vi "Main.vi"() -> ()   [LabVIEW 2026]
doc: "This Continuous Measurement sample project is based on the Queued Message Handler template.\n\nThe Event Handling Loop generates messages based on user interface actions.\n\nThe Message Handling Loop processes messages generated by the Event Handling Loop, or by other messages. There are also Acquisition and Logging message handling loop subVIs, and a chart updating loop."
uses:
  Settings/Settings.ctl
  Acquisition/Hardware Configuration.ctl
  Acquisition/Signal Type.ctl
  Logging/Logging Configuration.ctl
  controls/UI Data.ctl
  controls/UI State.ctl
  support/Message Queue/Enqueue Message (Single).vi
  support/Message Queue/Enqueue Message (Array).vi
  <vilib>/Utility/error.llb/Error Cluster From Error Code.vi
  <vilib>/ErrorRing/Error Ring.xnode
  Acquisition/Acquisition.lvlib
  Logging/Logging.lvlib
  Settings/Settings.lvlib
  support/User Event - Stop/User Event - Stop.lvlib
  support/Message Queue/Message Queue.lvlib
  Settings/Settings Dialog.vi
panel:
  out "Data":waveform(dbl)[](graph)
  in  "Settings":bool
  in  "Start":bool
  in  "Stop":bool
  out "Status":string
  in  "Exit":bool
  # "Continuous Measurement Data Logger"
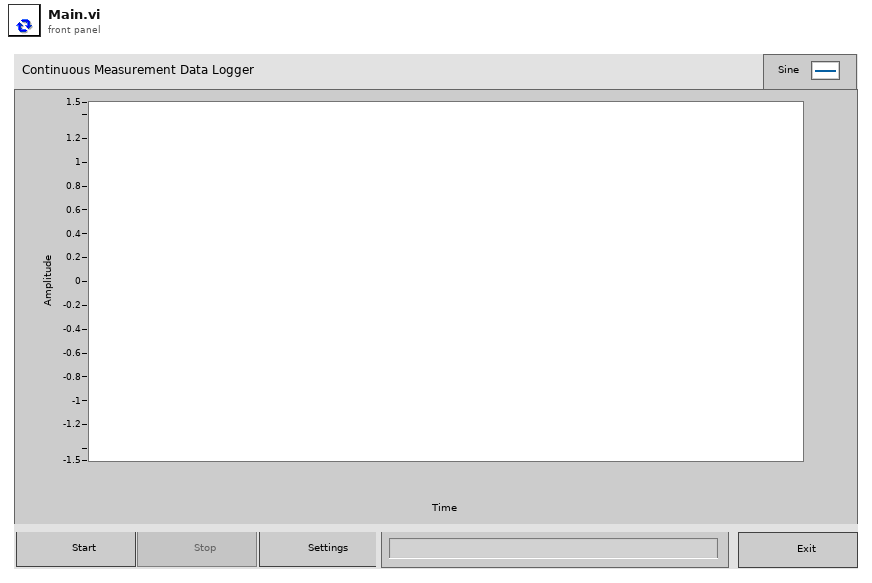
[diagram p1: front panel]
types:
  T1 = typedef "UI State.ctl" = enum16{"Idle", "Acquiring and Logging", "Waiting for Exit", "Waiting for Exit (Acq Stopped)", "Waiting for Exit (Log Stopped)", "Waiting for Stop", "Waiting for Stop (Acq Stopped)", "Waiting for Stop (Log Stopped)"}
  T2 = typedef "UI Data.ctl" = cluster{"Start Ref":refnum<vi>, "Stop Ref":refnum<vi>, "Settings Ref":refnum<vi>, "Exit Ref":refnum<vi>, "Status Ref":refnum<vi>, "Data Ref":refnum<vi>}
  T3 = typedef "Settings.lvlib/Settings.ctl" = cluster{"Hardware Configuration":T4, "Logging Configuration":T6}
  T4 = typedef "Acquisition.lvlib/Hardware Configuration.ctl" = cluster{"HW Refnum <Replace Me>":string, "Signal Type <Replace Me>":T5}
  T5 = typedef "Acquisition.lvlib/Signal Type.ctl" = enum16{"Sine Wave", "Square with Noise"}
  T6 = typedef "Logging.lvlib/Logging Configuration.ctl" = cluster{"Log File Base Path":path, "TDMS File Reference":refnum<k34>}
  T7 = typedef "Message Queue.lvlib/All Message Queues.ctl" = cluster{"UI":refnum<queue>, "Acquisition":refnum<queue>, "Logging":refnum<queue>}
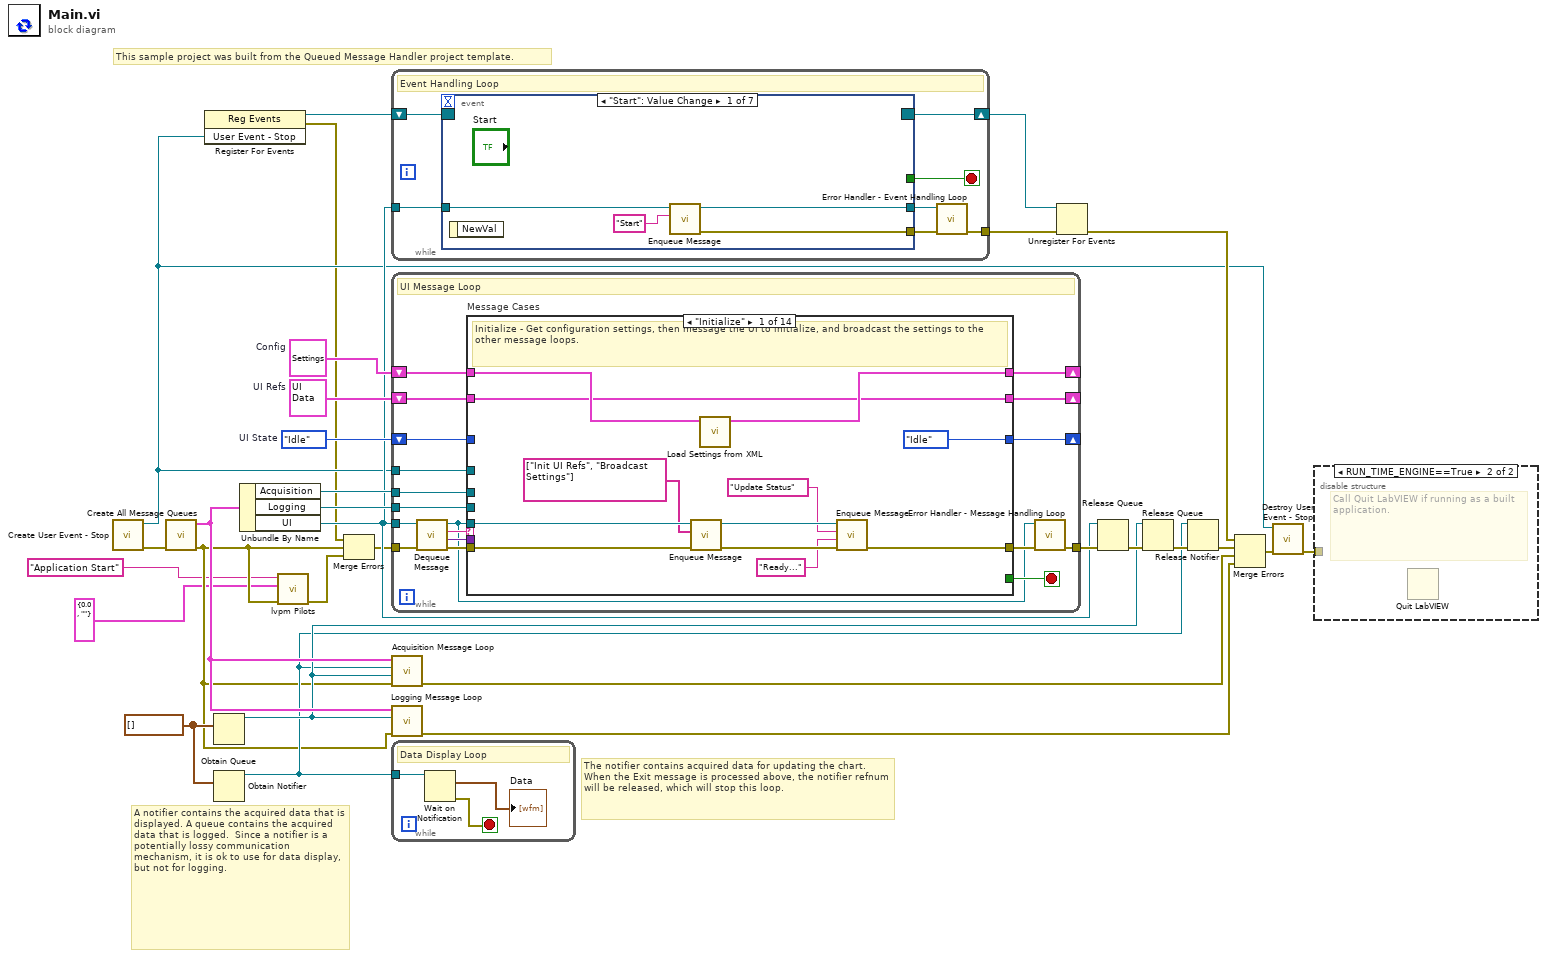
[diagram p0: block diagram]
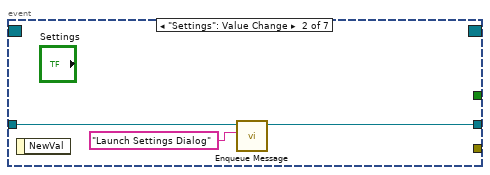
[diagram p3: hidden frame]
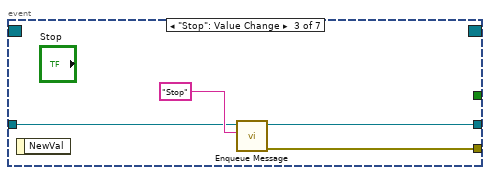
[diagram p4: hidden frame]
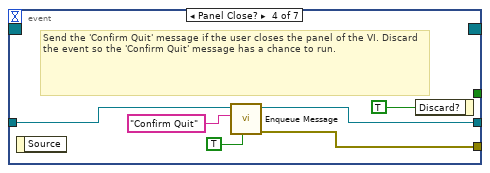
[diagram p5: hidden frame]
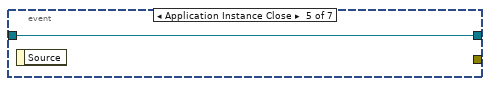
[diagram p6: hidden frame]
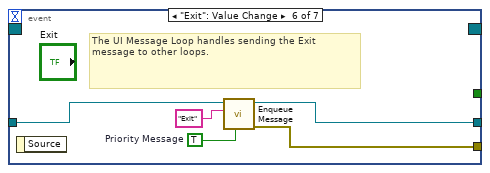
[diagram p7: hidden frame]
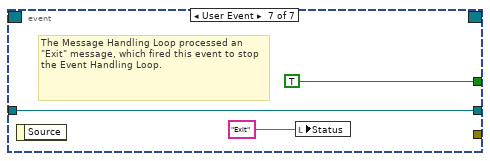
[diagram p8: hidden frame]
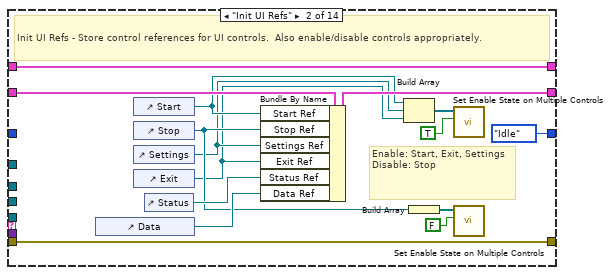
[diagram p9: hidden frame]
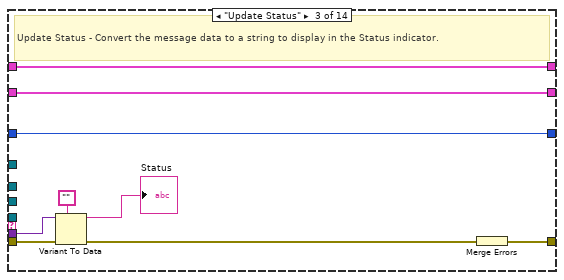
[diagram p10: hidden frame]
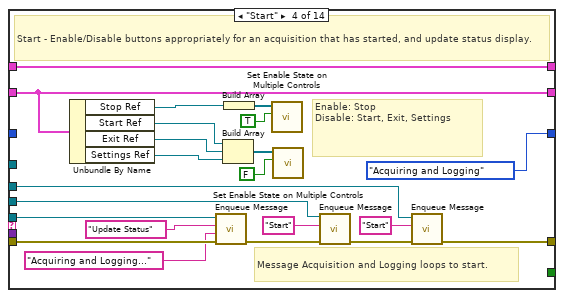
[diagram p11: hidden frame]
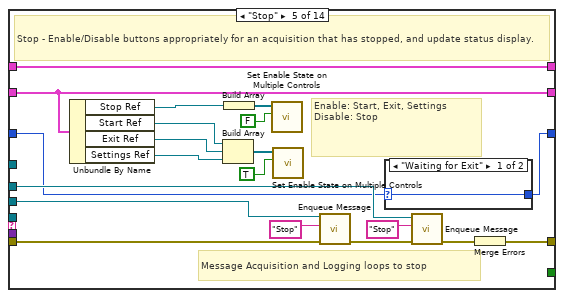
[diagram p12: hidden frame]
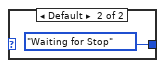
[diagram p13: hidden frame]
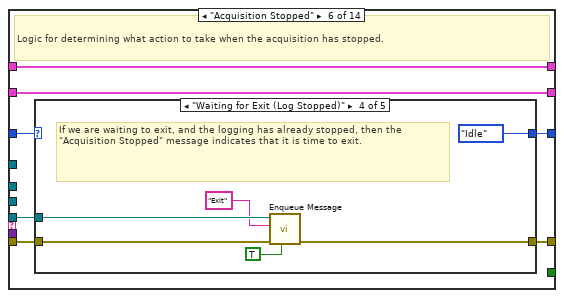
[diagram p14: hidden frame]
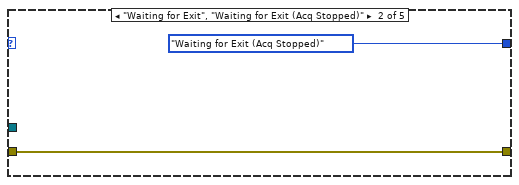
[diagram p16: hidden frame]
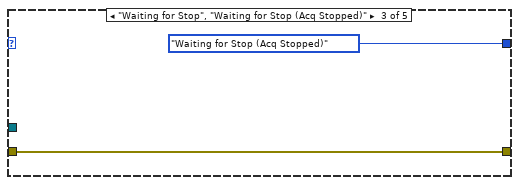
[diagram p17: hidden frame]
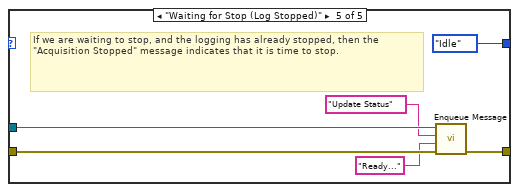
[diagram p18: hidden frame]
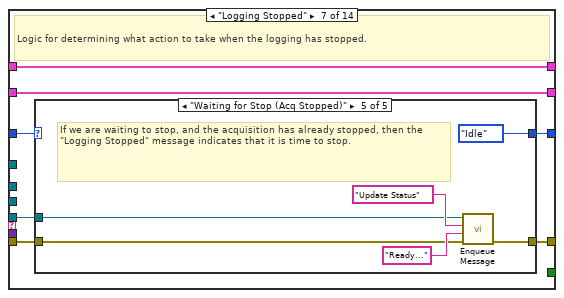
[diagram p19: hidden frame]
diagram:
  w18 = UI_State."Idle"  # UI State
  w9 = waveform(dbl)[] []
  w21 = T2 {"Start Ref"=refnum, "Stop Ref"=refnum, "Settings Ref"=refnum, "Exit Ref"=refnum, "Status Ref"=refnum, "Data Ref"=refnum}  # UI Refs
  w24 = T3 {"Hardware Configuration"={"HW Refnum <Replace Me>"="", "Signal Type <Replace Me>"=enum."Sine Wave"}, "Logging Configuration"={"Log File Base Path"=path "", "TDMS File Reference"=refnum}}  # Config
  # "This sample project was built from the Queued Message Handler project template."
  # "A notifier contains the acquired data that is displayed. A queue contains the acquired data that is logged.  Since a notifier is a potentially lossy communication mechanism, it is ok to use for data display, but not for logging."
  # "The notifier contains acquired data for updating the chart. When the Exit message is processed above, the notifier refnum will be released, which will stop this loop."
  n1 = call "Create User Event - Stop.vi"() -> ("error out"=w27:errorcluster, "User Event - Stop"=w7:refnum<user-event>)  [unwired: 10 in]
  n2 = call "Create All Message Queues.vi"("error in (no error)"=w27) -> ("error out"=w4:errorcluster, "Message Queues out"=w26:T7)  [unwired: 9 in]
  n3 = register-events(w7) -> (reference out=w8:refnum<event-registration>, error out=w5:errorcluster)  [unwired: 2 in]
  n4 = Obtain Queue(element data type=w9) -> (queue out=w11:refnum<queue>)  [unwired: 4 in, 2 out]
  n5 = Obtain Notifier(notification data type=w9) -> (notifier out=w10:refnum<notifier>)  [unwired: 3 in, 2 out]
  n6 = Unbundle By Name(w26) -> ("Acquisition"=w20:refnum<queue>, "Logging"=w19:refnum<queue>, "UI"=w16:refnum<queue>)
  n7 = call "lvpm Pilots.vi"("error in"=w4, "settings"=cluster{"rate (Hz)":dbl, "channel":string} {"rate (Hz)"=0.0, "channel"=""}, "message"="Application Start") -> ("error out"=w1:errorcluster)  [unwired: 7 in, 1 out]
  n8 = Merge Errors(w5, w4, w1) -> (w6:errorcluster)
  n9 = while {
    tunnel: w16 -> [w36]
    tunnel: [w33] -> w29
    shift-right: [w35] -> w22
    shift-left: w8 -> [w37]
    stop <- w34 stop-if-true
    # "Event Handling Loop"
    n10 = event shown="[0] \"Start\": Value Change" {
      selector: w37 -> [_ _ _ _ _ _ _]
      dyn-events: [_ _ _ _ _ _ _] -> w35
      timeout: _ -> [_ _ _ _ _ _ _]
      tunnel: [_ _ _ _ _ _ TRUE ("Discard?")] -> w34
      tunnel: w36 -> [w41 w43 w47 w52 w55 w57 w61]
      tunnel: [w39 _ w46 w50 _ w60 _] -> w32
      tunnel: [w38 w42 w45 w51 w55 w56 w61] -> w31
      event "Start": Value Change {
        n11 = event-data() -> ()  [unwired: 1 in, 1 out]
        n12 = call-poly "Enqueue Message.vi"("Message"="Start", "Message Queue"=w41) -> ("error out"=w39:errorcluster, "dup Message Queue"=w38:refnum<queue>)  [unwired: 8 in]
      }
      event "Settings": Value Change {
        n13 = event-data() -> ()  [unwired: 1 in, 1 out]
        n14 = call-poly "Enqueue Message.vi"("Message"="Launch Settings Dialog", "Message Queue"=w43) -> ("dup Message Queue"=w42:refnum<queue>)  [unwired: 8 in, 1 out]
      }
      event "Stop": Value Change {
        n15 = event-data() -> ()  [unwired: 1 in, 1 out]
        n16 = call-poly "Enqueue Message.vi"("Message"="Stop", "Message Queue"=w47) -> ("error out"=w46:errorcluster, "dup Message Queue"=w45:refnum<queue>)  [unwired: 8 in]
      }
      event Panel Close? {
        # "Send the 'Confirm Quit' message if the user closes the panel of the VI. Discard the event so the 'Confirm Quit' message has a chance to run."
        n17 = event-data() -> ()  [unwired: 1 in, 1 out]
        n18 = call-poly "Enqueue Message.vi"("Priority Message? (F)"=TRUE, "Message"="Confirm Quit", "Message Queue"=w52) -> ("error out"=w50:errorcluster, "dup Message Queue"=w51:refnum<queue>)  [unwired: 7 in]
        n19 = event-data("Discard?"=TRUE) -> ()  [unwired: 1 in, 1 out]
      }
      event Application Instance Close {
        n20 = event-data() -> ()  [unwired: 1 in, 1 out]
      }
      event "Exit": Value Change {
        w58 = TRUE  # Priority Message
        # "The UI Message Loop handles sending the Exit message to other loops."
        n21 = event-data() -> ()  [unwired: 1 in, 1 out]
        n22 = call-poly "Enqueue Message.vi"("Priority Message? (F)"=w58, "Message"="Exit", "Message Queue"=w57) -> ("error out"=w60:errorcluster, "dup Message Queue"=w56:refnum<queue>)  [unwired: 7 in]
      }
      event User Event {
        # "The Message Handling Loop processed an \"Exit\" message, which fired this event to stop the Event Handling Loop."
        n23 = event-data() -> ()  [unwired: 1 in, 1 out]
        n24 = local write "Status"("Exit" ("Exit String")) -> ()
      }
    }
    n25 = call "Error Handler - Event Handling Loop.vi"("error in (no error)"=w32, "Message Queue"=w31) -> ("dup error in"=w33:errorcluster)  [unwired: 8 in, 1 out]
  }
  n26 = while {
    tunnel: w16 -> [w75]
    tunnel: w7 -> [w80]
    shift-right: [w74] -> _
    shift-left: w24 -> [w73]
    shift-right: [w71] -> _
    shift-left: w21 -> [w72]
    tunnel: w20 -> [w70]
    tunnel: w19 -> [w69]
    shift-right: [w64] -> _
    shift-left: w18 -> [w65]
    tunnel: w6 -> [w79]
    tunnel: [w68] -> w30
    stop <- w81 stop-if-true
    # "UI Message Loop"
    n27 = call "Dequeue Message.vi"("error in (no error)"=w79, "Message Queue"=w75) -> ("error out"=w78:errorcluster, "Message Data"=w76:variant, "Message"=w77:string, "dup Message Queue"=w66:refnum<queue>)  [unwired: 6 in]
    n28 = case "Message Cases" shown="\"Initialize\"" w77 {
      selector: w77 -> [_ _ _ _ _ _ _ _ _ _ _ _ _ w296]
      tunnel: w66 -> [w86 _ _ w139 _ w164 w189 _ w228 _ w249 _ _ _]
      tunnel: w78 -> [w85 w108 w116 w138 w158 w165 w190 w217 w230 w237 w248 w277 w294 _]
      tunnel: [w82 w108 w117 w121 w159 w162 w187 w222 w223 w240 w247 w287 w293 w295] -> w67
      tunnel: [_ _ _ _ _ _ _ _ _ _ _ TRUE _ _] -> w81
      tunnel: w76 -> [_ _ w115 _ _ _ _ _ _ w241 _ w275 _ _]
      tunnel: w80 -> [_ _ _ _ _ _ _ _ _ _ _ w288 _ _]
      tunnel: [w92 w107 w111 w137 w157 w168 w193 w220 w227 w245 w252 w286 w292 w299] -> w74
      tunnel: w73 -> [w93 w107 w111 w137 w157 w168 w193 w220 w231 w245 w252 w286 w292 w299]
      tunnel: w72 -> [w87 w106 w110 w134 w156 w167 w192 w215 w225 w244 w251 w285 w291 w298]
      tunnel: [w87 w103 w110 w134 w156 w167 w192 w215 w225 w244 w251 w285 w291 w298] -> w71
      tunnel: w70 -> [_ _ _ w120 w143 _ _ w214 _ _ _ w284 _ _]
      tunnel: w69 -> [_ _ _ w123 w146 _ _ w213 _ _ _ w283 _ _]
      tunnel: w65 -> [_ _ w109 _ w140 w166 w191 w212 w224 w239 w250 _ w290 w297]
      tunnel: [UI_State."Idle" ("UI State") UI_State."Idle" ("UI State") w109 UI_State."Acquiring and Logging" ("UI State") w141 w163 w188 w212 w224 w239 w246 UI_State."Idle" ("UI State") w290 w297] -> w64
      frame "Initialize" {
        # "Initialize - Get configuration settings, then message the UI to initialize, and broadcast the settings to the other message loops."
        n29 = call-poly "Enqueue Message.vi"("error in (no error)"=w85, "Message Array"=string[] ["Init UI Refs", "Broadcast Settings"], "Message Queue"=w86) -> ("error out"=w91:errorcluster, "dup Message Queue"=w90:refnum<queue>)  [unwired: 7 in]
        n30 = call "Load Settings from XML.vi"("Settings in"=w93) -> ("Settings out"=w92:T3)  [unwired: 9 in, 1 out]
        n31 = call-poly "Enqueue Message.vi"("error in (no error)"=w91, "Message Data"="Ready..." ("Ready..."), "Message"="Update Status", "Message Queue"=w90) -> ("error out"=w82:errorcluster)  [unwired: 6 in, 1 out]
      }
      frame "Init UI Refs" {
        # "Enable: Start, Exit, Settings\nDisable: Stop"
        # "Init UI Refs - Store control references for UI controls.  Also enable/disable controls appropriately."
        n32 = control-ref of="Data"() -> (w104:refnum<vi>)
        n33 = control-ref of="Start"() -> (w97:refnum<vi>)
        n34 = control-ref of="Stop"() -> (w98:refnum<vi>)
        n35 = control-ref of="Settings"() -> (w96:refnum<vi>)
        n36 = control-ref of="Exit"() -> (w95:refnum<vi>)
        n37 = control-ref of="Status"() -> (w105:refnum<vi>)
        n38 = Bundle By Name(cluster=w106, "Start Ref"=w97, "Stop Ref"=w98, "Settings Ref"=w96, "Exit Ref"=w95, "Status Ref"=w105, "Data Ref"=w104) -> (w103:T2)
        n39 = Build Array(w97, w96, w95) -> (w101:refnum<vi>[])
        n40 = Build Array(w98) -> (w100:refnum<vi>[])
        n41 = call "Set Enable State on Multiple Controls.vi"("Enable?"=TRUE, "Controls"=w101) -> ()  [unwired: 10 in]
        n42 = call "Set Enable State on Multiple Controls.vi"("Enable?"=FALSE, "Controls"=w100) -> ()  [unwired: 10 in]
      }
      frame "Update Status" {
        # "Update Status - Convert the message data to a string to display in the Status indicator."
        n43 = Variant To Data(error in=w116, type="", Variant=w115) -> (data=→"Status":string, error out=w113:errorcluster)
        n44 = Merge Errors(w113) -> (w117:errorcluster)
      }
      frame "Start" {
        # "Message Acquisition and Logging loops to start."
        # "Enable: Stop\nDisable: Start, Exit, Settings"
        # "Start - Enable/Disable buttons appropriately for an acquisition that has started, and update status display."
        n45 = Unbundle By Name(w134) -> ("Stop Ref"=w129:refnum<vi>, "Start Ref"=w128:refnum<vi>, "Exit Ref"=w127:refnum<vi>, "Settings Ref"=w126:refnum<vi>)
        n46 = call-poly "Enqueue Message.vi"("error in (no error)"=w138, "Message Data"="Acquiring and Logging..." ("Acquiring and Logging..."), "Message"="Update Status", "Message Queue"=w139) -> ("error out"=w125:errorcluster)  [unwired: 6 in, 1 out]
        n47 = Build Array(w128, w127, w126) -> (w132:refnum<vi>[])
        n48 = Build Array(w129) -> (w131:refnum<vi>[])
        n49 = call "Set Enable State on Multiple Controls.vi"("Enable?"=TRUE, "Controls"=w131) -> ()  [unwired: 10 in]
        n50 = call "Set Enable State on Multiple Controls.vi"("Enable?"=FALSE, "Controls"=w132) -> ()  [unwired: 10 in]
        n51 = call-poly "Enqueue Message.vi"("error in (no error)"=w125, "Message"="Start", "Message Queue"=w123) -> ("error out"=w122:errorcluster)  [unwired: 7 in, 1 out]
        n52 = call-poly "Enqueue Message.vi"("error in (no error)"=w122, "Message"="Start", "Message Queue"=w120) -> ("error out"=w121:errorcluster)  [unwired: 7 in, 1 out]
      }
      frame "Stop" {
        # "Message Acquisition and Logging loops to stop"
        # "Enable: Start, Exit, Settings\nDisable: Stop"
        # "Stop - Enable/Disable buttons appropriately for an acquisition that has stopped, and update status display."
        n53 = Unbundle By Name(w156) -> ("Stop Ref"=w151:refnum<vi>, "Start Ref"=w150:refnum<vi>, "Exit Ref"=w149:refnum<vi>, "Settings Ref"=w148:refnum<vi>)
        n54 = Build Array(w150, w149, w148) -> (w154:refnum<vi>[])
        n55 = Build Array(w151) -> (w153:refnum<vi>[])
        n56 = call "Set Enable State on Multiple Controls.vi"("Enable?"=FALSE, "Controls"=w153) -> ()  [unwired: 10 in]
        n57 = call "Set Enable State on Multiple Controls.vi"("Enable?"=TRUE, "Controls"=w154) -> ()  [unwired: 10 in]
        n58 = call-poly "Enqueue Message.vi"("error in (no error)"=w158, "Message"="Stop", "Message Queue"=w146) -> ("error out"=w145:errorcluster)  [unwired: 7 in, 1 out]
        n59 = case shown="\"Waiting for Exit\"" w140 {
          selector: w140 -> [w160 _]
          tunnel: [w160 UI_State."Waiting for Stop" ("UI State")] -> w141
          frame "Waiting for Exit" {
          }
          frame Default {
          }
        }
        n60 = call-poly "Enqueue Message.vi"("error in (no error)"=w145, "Message"="Stop", "Message Queue"=w143) -> ("error out"=w144:errorcluster)  [unwired: 7 in, 1 out]
        n61 = Merge Errors(w144) -> (w159:errorcluster)
      }
      frame "Acquisition Stopped" {
        # "Logic for determining what action to take when the acquisition has stopped."
        n62 = case shown="\"Waiting for Exit (Log Stopped)\"" w166 {
          selector: w166 -> [w170 _ _ _ _]
          tunnel: w165 -> [w169 w172 w174 w180 w186]
          tunnel: w164 -> [_ _ _ w178 w183]
          tunnel: [w170 UI_State."Waiting for Exit (Acq Stopped)" ("UI State") UI_State."Waiting for Stop (Acq Stopped)" ("UI State") UI_State."Idle" ("UI State") UI_State."Idle" ("UI State")] -> w163
          tunnel: [w169 w172 w174 w179 w184] -> w162
          frame Default {
          }
          frame "Waiting for Exit", "Waiting for Exit (Acq Stopped)" {
          }
          frame "Waiting for Stop", "Waiting for Stop (Acq Stopped)" {
          }
          frame "Waiting for Exit (Log Stopped)" {
            # "If we are waiting to exit, and the logging has already stopped, then the \"Acquisition Stopped\" message indicates that it is time to exit."
            n63 = call-poly "Enqueue Message.vi"("Priority Message? (F)"=TRUE, "error in (no error)"=w180, "Message"="Exit", "Message Queue"=w178) -> ("error out"=w179:errorcluster)  [unwired: 6 in, 1 out]
          }
          frame "Waiting for Stop (Log Stopped)" {
            # "If we are waiting to stop, and the logging has already stopped, then the \"Acquisition Stopped\" message indicates that it is time to stop."
            n64 = call-poly "Enqueue Message.vi"("error in (no error)"=w186, "Message Data"="Ready..." ("Ready..."), "Message"="Update Status", "Message Queue"=w183) -> ("error out"=w184:errorcluster)  [unwired: 6 in, 1 out]
          }
        }
      }
      frame "Logging Stopped" {
        # "Logic for determining what action to take when the logging has stopped."
        n65 = case shown="\"Waiting for Stop (Acq Stopped)\"" w191 {
          selector: w191 -> [w195 _ _ _ _]
          tunnel: w190 -> [w194 w197 w199 w205 w208]
          tunnel: w189 -> [_ _ _ w203 w207]
          tunnel: [w195 UI_State."Waiting for Exit (Log Stopped)" ("UI State") UI_State."Waiting for Stop (Log Stopped)" ("UI State") UI_State."Idle" ("UI State") UI_State."Idle" ("UI State")] -> w188
          tunnel: [w194 w197 w199 w204 w206] -> w187
          frame Default {
          }
          frame "Waiting for Exit", "Waiting for Exit (Log Stopped)" {
          }
          frame "Waiting for Stop", "Waiting for Stop (Log Stopped)" {
          }
          frame "Waiting for Exit (Acq Stopped)" {
            # "If we are waiting to exit, and the acquisition has already stopped, then the \"Logging Stopped\" message indicates that it is time to exit."
            n66 = call-poly "Enqueue Message.vi"("Priority Message? (F)"=TRUE, "error in (no error)"=w205, "Message"="Exit", "Message Queue"=w203) -> ("error out"=w204:errorcluster)  [unwired: 6 in, 1 out]
          }
          frame "Waiting for Stop (Acq Stopped)" {
            # "If we are waiting to stop, and the acquisition has already stopped, then the \"Logging Stopped\" message indicates that it is time to stop."
            n67 = call-poly "Enqueue Message.vi"("error in (no error)"=w208, "Message Data"="Ready..." ("Ready..."), "Message"="Update Status", "Message Queue"=w207) -> ("error out"=w206:errorcluster)  [unwired: 6 in, 1 out]
          }
        }
      }
      frame "Broadcast settings" {
        w216 = "Update Settings" ("Message")
        # "Broadcast settings - Send the 'Update Settings' message to the Logging and Acquisition message loops."
        n68 = Unbundle By Name(w220) -> ("Logging Configuration"=w219:T6)  [unwired: 1 out]
        n69 = call-poly "Enqueue Message.vi"("Message"=w216, "Message Queue"=w214) -> ("error out"=w221:errorcluster)  [unwired: 8 in, 1 out]
        n70 = call-poly "Enqueue Message.vi"("error in (no error)"=w221, "Message Data"=w219, "Message"=w216, "Message Queue"=w213) -> ("error out"=w218:errorcluster)  [unwired: 6 in, 1 out]
        n71 = Merge Errors(w218, w217) -> (w222:errorcluster)
      }
      frame "Launch Settings Dialog" {
        # "Launch Settings Dialog - Launch the Settings Dialog when the user clicks the 'Settings' button."
        n72 = call-by-ref "?"("error in (no error)"=w230, "Settings in"=w231) -> ("error out"=w226:errorcluster, "Cancelled?"=w229:bool, "Settings out"=w227:T3)  [unwired: 8 in, 3 out]
        n73 = case shown="False" w229 {
          tunnel: w228 -> [w235 _]
          tunnel: w226 -> [w234 w236]
          tunnel: [w233 w236] -> w223
          frame False {
            n74 = call-poly "Enqueue Message.vi"("error in (no error)"=w234, "Message"="Broadcast Settings", "Message Queue"=w235) -> ("error out"=w233:errorcluster)  [unwired: 7 in, 1 out]
          }
          frame True {
          }
        }
      }
      frame "Error" {
        # "Error - Display an error dialog. This message is sent by the \"Error Handler\" VIs at the end of other loops in this application."
        n75 = Variant To Data(error in=w237, type=errorcluster {"status"=FALSE, "code"=0, "source"=""} ("error constant"), Variant=w241) -> (data=w238:errorcluster, error out=w242:errorcluster)
        n76 = call <vilib>:"Simple Error Handler.vi"("error in (no error)"=w238) -> ()  [unwired: 4 in, 5 out]
        n77 = Merge Errors(w242) -> (w240:errorcluster)
      }
      frame "Confirm Quit" {
        # "Confirm Quit - Message that can confirm whether or not the user wants to exit the application."
        n78 = case shown="\"Acquiring and Logging\"" w250 {
          tunnel: w249 -> [w258 w262]
          tunnel: w248 -> [w257 w261]
          tunnel: [w256 w260] -> w247
          tunnel: [UI_State."Idle" ("UI State") w259] -> w246
          frame Default {
            # "If 'Confirm Quit' comes in while the system is idle, there is no need for a confirmation message."
            n79 = call-poly "Enqueue Message.vi"("Priority Message? (F)"=TRUE, "error in (no error)"=w257, "Message"="Exit", "Message Queue"=w258) -> ("error out"=w256:errorcluster)  [unwired: 6 in, 1 out]
          }
          frame "Acquiring and Logging" {
            n80 = Two Button Dialog(message="Are you sure you want to quit while the acquisition is running?" ("Confirm Quit Message"), 1:"No" ("No"), 2:"Yes" ("Yes")) -> (T button?=w263:bool)
            n81 = case shown="True" w263 {
              tunnel: w262 -> [_ w272]
              tunnel: w261 -> [w268 w273]
              tunnel: [w268 w271] -> w260
              tunnel: [UI_State."Acquiring and Logging" ("UI State") UI_State."Waiting for Exit" ("UI State")] -> w259
              frame False {
                # "User did not want to quit."
              }
              frame True {
                n82 = call-poly "Enqueue Message.vi"("error in (no error)"=w273, "Message"="Stop", "Message Queue"=w272) -> ("error out"=w271:errorcluster)  [unwired: 7 in, 1 out]
              }
            }
          }
        }
      }
      frame "Exit" {
        w279 = TRUE ("Priority Message? (F)")
        w280 = "Exit" ("Message")
        # "Popup an error dialog if 'Exit' was called as a result of an error."
        # "Stop the VI"
        # "Exit - Send Exit messages to the Acquisition and Logging loops, and fire the user event to stop the Event Handling Loop."
        n83 = Variant To Data(type=errorcluster {"status"=FALSE, "code"=0, "source"=""} ("error constant"), Variant=w275) -> (data=w274:errorcluster)  [unwired: 1 in, 1 out]
        n84 = call <vilib>:"Simple Error Handler.vi"("error in (no error)"=w274) -> ()  [unwired: 4 in, 5 out]
        n85 = call-poly "Enqueue Message.vi"("Priority Message? (F)"=w279, "error in (no error)"=w277, "Message"=w280, "Message Queue"=w284) -> ("error out"=w281:errorcluster)  [unwired: 6 in, 1 out]
        n86 = call-poly "Enqueue Message.vi"("Priority Message? (F)"=w279, "error in (no error)"=w281, "Message"=w280, "Message Queue"=w283) -> ("error out"=w278:errorcluster)  [unwired: 6 in, 1 out]
        n87 = call "Fire User Event - Stop.vi"("error in (no error)"=w278, "User Event - Stop"=w288) -> ("error out"=w287:errorcluster)  [unwired: 9 in]
      }
      frame "---Copy This Frame---" {
        # "Duplicate this frame when creating new messages.  Change this comment in the duplicated frame to describe this message."
        n88 = Merge Errors(w294) -> (w293:errorcluster)
      }
      frame Default {
        # "'Default' case only runs if there is a message that isn't defined in any of the other cases.  Output a programming error."
        n89 = xnode "Error Ring"("parameter 0"=w296) -> ("error out"=w295:errorcluster)
      }
    }
    n90 = call "Error Handler - Message Handling Loop.vi"("error in (no error)"=w67, "Message Queue"=w66) -> ("dup error in"=w68:errorcluster)  [unwired: 8 in, 1 out]
  }
  n91 = call "Acquisition Message Loop.vi"("error in (no error)"=w4, "Data Queue"=w11, "Data Notifier"=w10, "Message Queues"=w26) -> ("error out"=w28:errorcluster)  [unwired: 7 in]
  n92 = call "Logging Message Loop.vi"("error in (no error)"=w4, "Data Queue"=w11, "Message Queues"=w26) -> ("error out"=w25:errorcluster)  [unwired: 8 in]
  n93 = while "Data Display Loop" {
    tunnel: w10 -> [w309]
    stop <- w307 stop-if-true
    # "Data Display Loop"
    n94 = Wait on Notification(notifier=w309) -> (notification=→"Data":waveform(dbl)[], error out=w307:errorcluster)  [unwired: 3 in, 2 out]
  }
  n95 = Unregister For Events(event registration refnum=w22, error in=w29) -> (error out=w23:errorcluster)
  n96 = Release Queue(queue=w16, error in (no error)=w30) -> (error out=w14:errorcluster)  [unwired: 1 in, 2 out]
  n97 = Release Queue(queue=w11, error in (no error)=w14) -> (error out=w13:errorcluster)  [unwired: 1 in, 2 out]
  n98 = Release Notifier(notifier=w10, error in (no error)=w13) -> (error out=w12:errorcluster)  [unwired: 1 in, 2 out]
  n99 = Merge Errors(w23, w12, w28, w25) -> (w17:errorcluster)
  n100 = call "Destroy User Event - Stop.vi"("error in (no error)"=w17, "User Event - Stop"=w7) -> ("error out"=w15:errorcluster)  [unwired: 9 in]
  n101 = disable-structure shown="RUN_TIME_ENGINE==True" {
    disable-tunnel: w15 -> [_ _]
    frame condition #0 (active) {
    }
    frame condition #1 {
      # "Call Quit LabVIEW if running as a built application."
      n102 = Quit LabVIEW() -> ()  [unwired: 1 in]
    }
  }
